vi "Modify window front.vi"(5 "Left":i16, 7 "Top":i16, 8 "error in":errorcluster, 9 "Right":i16, 10 "Bottom":i16, 11 "Module ID":i32=-1) -> (0 "error out":errorcluster)   [LabVIEW 2018, in "Popup.lvlib"]
doc: "修改窗口大小\n\n_____\nCreated using DQMH Framework: Event Scripter 7.1.1.1528."
uses:
  Popup.lvlib
  Modify window front Argument--cluster.ctl
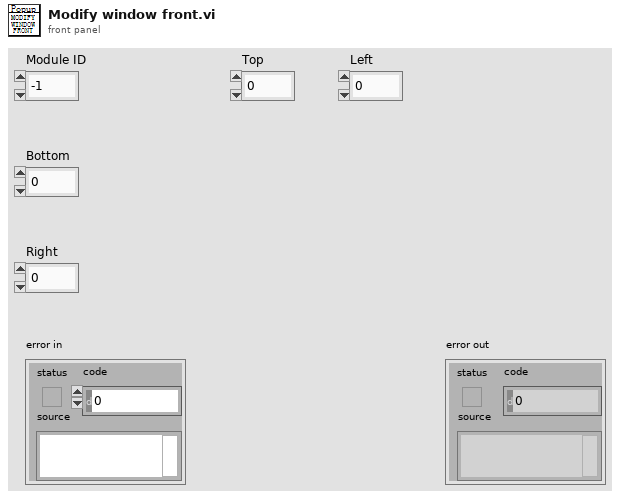
[diagram p1: front panel]
types:
  T1 = typedef "Popup.lvlib/Modify window front Argument--cluster.ctl" = cluster{"Module ID":i32, "Bottom":i16, "Right":i16, "Top":i16, "Left":i16}
  T2 = typedef "Popup.lvlib/Request Events--cluster.ctl" = cluster{"Stop Module":refnum<user-event>, "Show Panel":refnum<user-event>, "Hide Panel":refnum<user-event>, "Show Diagram":refnum<user-event>, "Get Module Execution Status":refnum<user-event>, "Change Panel":refnum<user-event>, "modify panl  origin position":refnum<user-event>, "Modify window front":refnum<user-event>, "Modify Title name":refnum<user-event>}
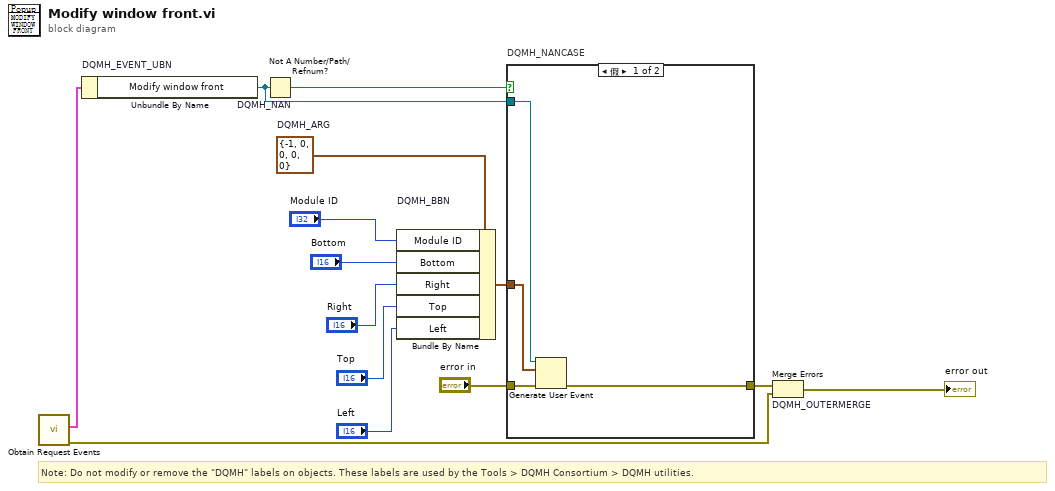
[diagram p0: block diagram]
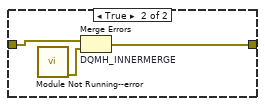
[diagram p2: hidden frame]
diagram:
  w8 = T1 {"Module ID"=-1, "Bottom"=0, "Right"=0, "Top"=0, "Left"=0}  # DQMH_ARG
  # "Note: Do not modify or remove the \"DQMH\" labels on objects. These labels are used by the Tools > DQMH Consortium > DQMH utilities."
  n1 = call "Obtain Request Events.vi"() -> ("error out"=w2:errorcluster, "Popup Request Events"=w1:T2)  [unwired: 10 in]
  n2 = Unbundle By Name "DQMH_EVENT_UBN"(w1) -> ("Modify window front"=w10:refnum<user-event>)
  n3 = Not A Number/Path/Refnum? "DQMH_NAN"(number/path/refnum=w10) -> (NaN/Path/Refnum?=w11:bool)
  n4 = Bundle By Name "DQMH_BBN"(cluster=w8, "Module ID"="Module ID", "Bottom"="Bottom", "Right"="Right", "Top"="Top", "Left"="Left") -> (w12:T1)
  n5 = case "DQMH_NANCASE" shown="假" w11 {
    tunnel: "error in" -> [w18 w21]
    tunnel: [w17 w20] -> w9
    tunnel: w10 -> [w16 _]
    tunnel: w12 -> [w15 _]
    frame False {
      n6 = Generate User Event(user event=w16, event data cluster=w15, error in=w18) -> (error out=w17:errorcluster)  [unwired: 1 in, 1 out]
    }
    frame True {
      n7 = call "Module Not Running--error.vi"() -> ("error out"=w19:errorcluster)  [unwired: 11 in]
      n8 = Merge Errors "DQMH_INNERMERGE"(w21, w19) -> (w20:errorcluster)
    }
  }
  n9 = Merge Errors "DQMH_OUTERMERGE"(w9, w2) -> (→"error out":errorcluster)
